vi "Explain Error (Improved) UI.vi"(8 "User VI Ref":refnum<vi>, 9 "Error Cluster":errorcluster) -> ()   [LabVIEW 2020, in "Explain Error Improved Dialog.lvlib"]
uses:
  Explain Error Improved Dialog/Explain Error Improved Dialog.lvlib
  <vilib>/Utility/error.llb/DialogTypeEnum.ctl
  <vilib>/Utility/error.llb/DialogType.ctl
  fc0d4d85-7f14-4b45-b7f8-c4820347555e.vi
  <vilib>/Platform/browser.llb/Open URL in Default Browser (string).vi
  <vilib>/Utility/inputDevices.llb/mouseAcquire.vi
  <vilib>/Utility/inputDevices.llb/keyboardAcquire.vi
  <vilib>/Utility/cursorutil.llb/Set Cursor (Icon Pict).vi
  <vilib>/Utility/inputDevices.llb/closeKeyboard.vi
  <vilib>/Utility/inputDevices.llb/closeMouse.vi
panel:
  in  "search google":bool
  out "Explanation":string
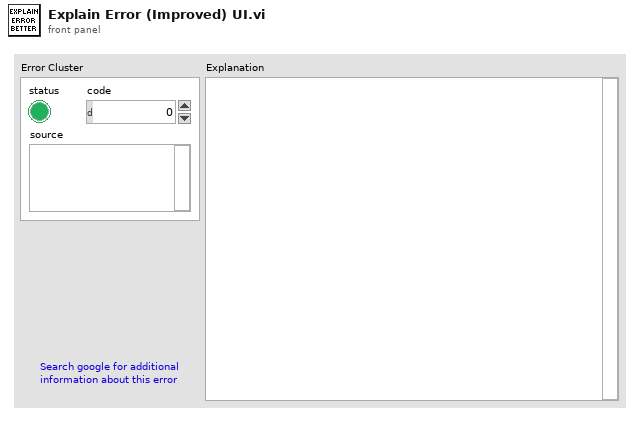
[diagram p1: front panel]
types:
  T1 = typedef "DialogTypeEnum.ctl" = enum16{"no dialog", "OK message", "continue or stop message", "auto error handling dialog", "OK message + warnings", "continue/stop + warnings"}
  T2 = typedef "DialogType.ctl" = u16
  T3 = cluster{"vi name":string, "start":i32, "end":i32}[]
  T4 = typedef "LVPoint32TypeDef.ctl" = cluster{"Horizontal":i32, "Vertical":i32}
  T5 = cluster{"button 1":bool, "button 2":bool, "button 3":bool, "button 4":bool}
  T6 = cluster{"vi name":string, "start":i32, "end":i32}
  T7 = enum16{"0", "1", "2", "3", "4", "5", "6", "7", "8", "9", "A", "B", "C", "D", "E", "F", "G", "H", "I", "J", "K", "L", "M", "N", "O", "P", "Q", "R", "S", "T", "U", "V", "W", "X", "Y", "Z", "F1", "F2", "F3", "F4", "F5", "F6", "F7", "F8", "F9", "F10", "F11", "F12", "F13", "F14", "F15", "ADD", "BACK", "BACKSLASH", "CAPITAL", "COMMA", "DECIMAL", "DELETE", "DIVIDE", "DOWN", "END", "EQUALS", "ESCAPE", "GRAVE (`)", "HOME", "INSERT", "LBRACKET", "LCONTROL", "LEFT", "L ALT", "LSHIFT", "LWIN", "MINUS", "MULTIPLY", "NEXT", "NUMLOCK", "NUMPAD_0", "NUMPAD_1", "NUMPAD_2", "NUMPAD_3", "NUMPAD_4", "NUMPAD_5", "NUMPAD_6", "NUMPAD_7", "NUMPAD_8", "NUMPAD_9", "PAUSE", "PERIOD", "PRIOR (PG UP)", "RBRACKET", "RCONTROL", "RETURN", "RIGHT", "R ALT", "RSHIFT", "RWIN", "SCROLL", "SEMICOLON", "SLASH", "SPACE", "SUBTRACT", "TAB", "UP", "ENTER (num pad)", "' (quote)"}[]
  T8 = cluster{"Shift":bool, "Ctrl":bool, "Alt":bool, "Cmd":bool, "Opt":bool}
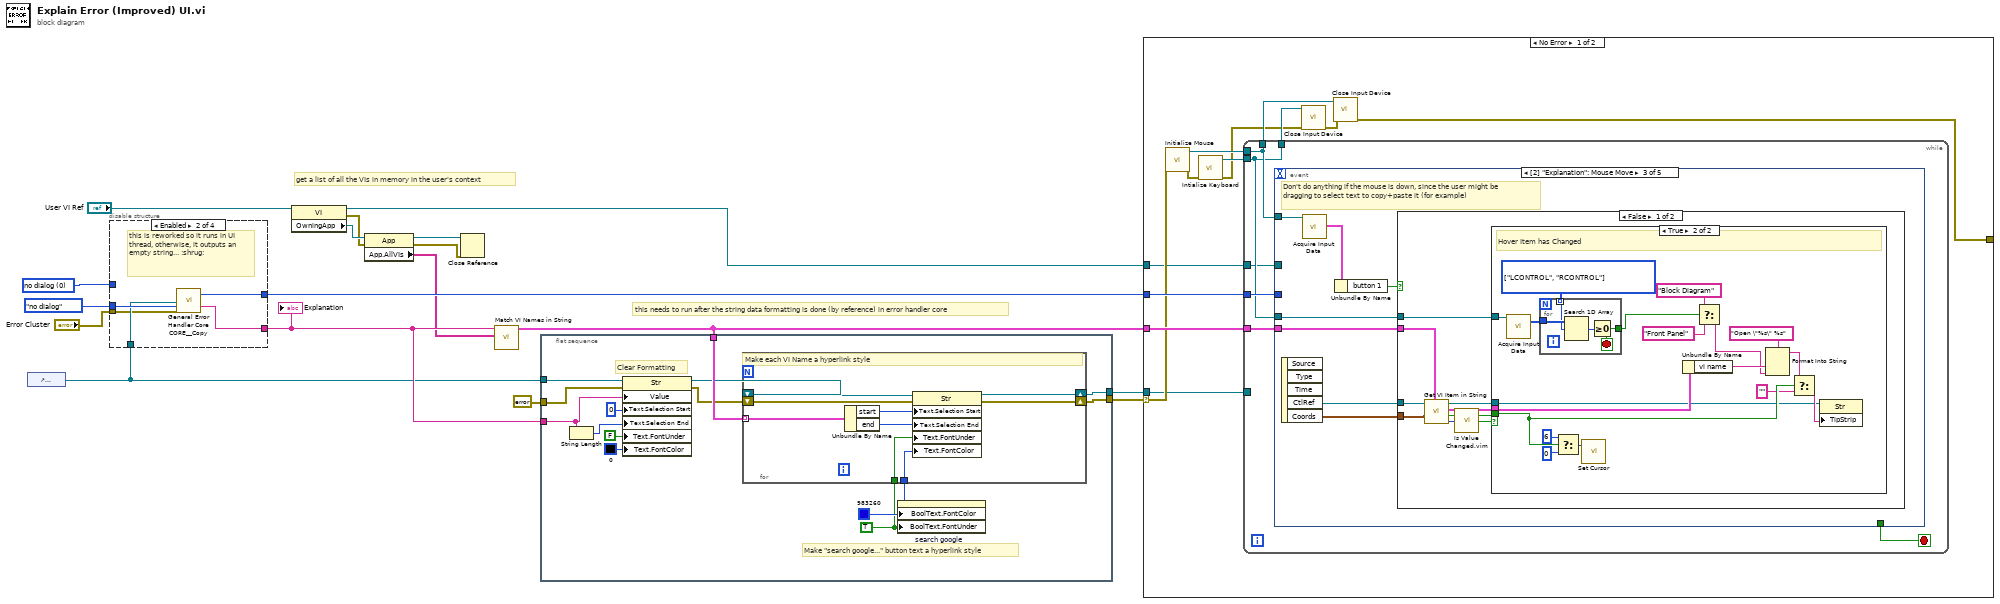
[diagram p0: block diagram]
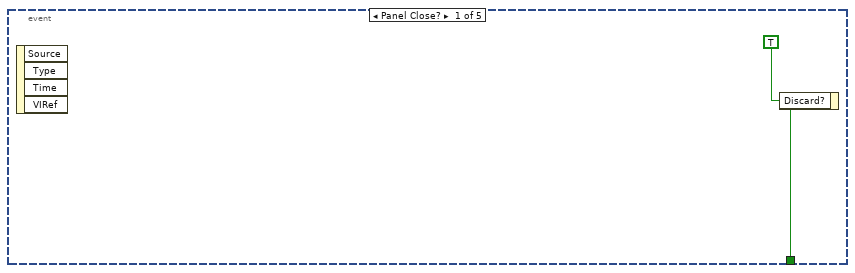
[diagram p2: hidden frame]
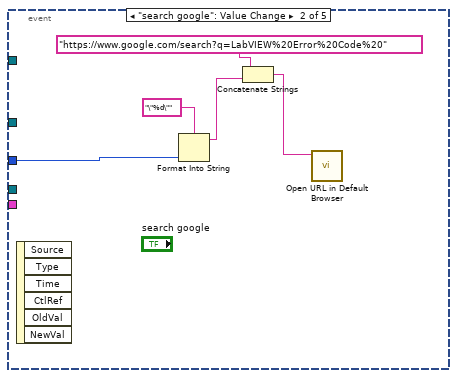
[diagram p3: hidden frame]
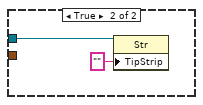
[diagram p5: hidden frame]
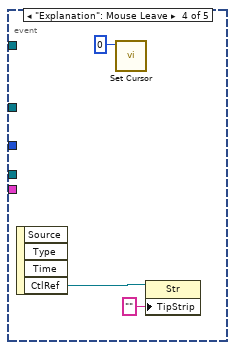
[diagram p6: hidden frame]
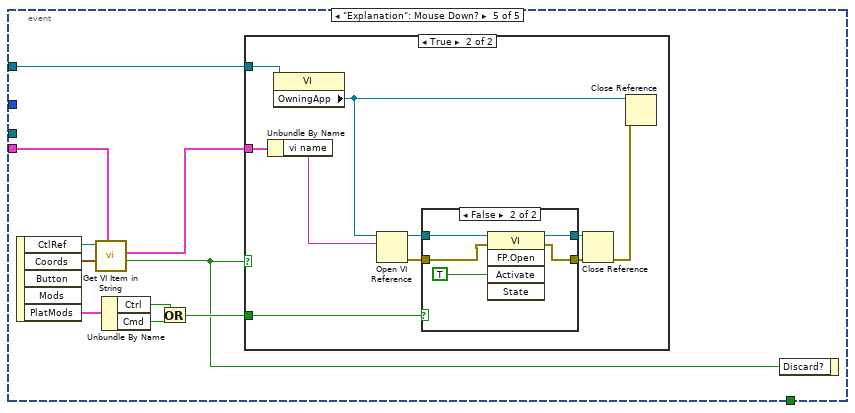
[diagram p7: hidden frame]
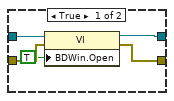
[diagram p9: hidden frame]
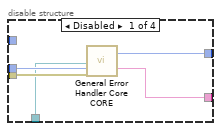
[diagram p11: hidden frame]
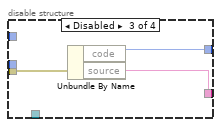
[diagram p12: hidden frame]
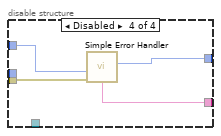
[diagram p13: hidden frame]
diagram:
  w12 = T2 0 items=["no dialog", "OK message", "continue or stop message", "OK message + warnings", "continue/stop + warnings"] ("type of dialog (OK msg:1)")
  # "this needs to run after the string data formatting is done (by reference) in error handler core"
  # "get a list of all the VIs in memory in the user's context"
  n1 = control-ref of="Explanation"() -> (w9:refnum<vi>)
  n2 = disable-structure shown="Enabled" {
    disable-tunnel: "Error Cluster" -> [w22 w23 w30 w34]
    disable-tunnel: DialogTypeEnum."no dialog" ("type of dialog (OK msg:1)") -> [w21 w27 _ _]
    disable-tunnel: [w19 w26 w28 w33] -> w10
    disable-tunnel: [w18 w25 w29 w32] -> w14
    disable-tunnel: w12 -> [_ _ _ w31]
    disable-tunnel: w9 -> [w20 w24 _ _]
    frame Disabled {
      n3 = call <vilib>:"General Error Handler Core CORE.vi"("String to Format (not a refnum)"=w20, "type of dialog (OK msg:1)"=w21, "error in (no error)"=w22) -> ("code out"=w18:i32, "message"=w19:string)  [unwired: 11 in, 4 out]
    }
    frame Enabled {
      # "this is reworked so it runs in UI thread, otherwise, it outputs an empty string... :shrug:"
      n4 = call "General Error Handler Core CORE__Copy.vi"("String to Format (not a refnum)"=w24, "type of dialog (OK msg:1)"=w27, "error in (no error)"=w23) -> ("code out"=w25:i32, "message"=w26:string)  [unwired: 11 in, 4 out]
    }
    frame Disabled {
      n5 = Unbundle By Name(w30) -> ("code"=w29:i32, "source"=w28:string)
    }
    frame Disabled {
      n6 = call <vilib>:"Simple Error Handler.vi"("type of dialog (OK msg:1)"=w31, "error in (no error)"=w34) -> ("code out"=w32:i32, "message"=w33:string)  [unwired: 3 in, 3 out]
    }
  }
  "Explanation" <- w10
  n7 = property class="VI"(reference="User VI Ref") -> (reference out=w7:refnum<vi>, error out=w3:errorcluster, "OwningApp"=w6:refnum<vi>)  [unwired: 1 in]
  n8 = property class="App"(reference=w6, error in=w3) -> (reference out=w4:refnum<vi>, error out=w2:errorcluster, "App.AllVIs"=w5:string[])
  n9 = Close Reference(reference=w4, error in (no error)=w2) -> ()  [unwired: 1 out]
  n10 = call "Match VI Names in String.vi"("Application:All VIs In Memory"=w5, "string"=w10) -> ("vi names"=w17:T3)  [unwired: 9 in]
  n11 = flat-sequence {
    tunnel: w17 -> [w48]
    tunnel: [w47] -> w16
    tunnel: w10 -> [w46]
    tunnel: w9 -> [w45]
    tunnel: [w44] -> w8
    tunnel: errorcluster {"status"=FALSE, "code"=0, "source"=""} ("error out") -> [w43]
    frame #0 {
      w38 = TRUE ("Text.Font:Underline")
      w39 = u32 983260
      # "Make \"search google...\" button text a hyperlink style"
      # "Clear Formatting"
      n12 = String Length(string=w46) -> (length=w37:i32)
      n13 = property class="Str"(reference=w45, error in=w43, "Value"=w46, "Text.Selection Start"=u32 0 ("Text.Selection:Start"), "Text.Selection End"=w37, "Text.FontUnder"=FALSE ("Text.Font:Underline"), "Text.FontColor"=u32 0 ("Text.Font:Color")) -> (reference out=w42:refnum<vi>, error out=w35:errorcluster)
      n14 = for {
        tunnel: w48 -> [w56] mode=indexing
        shift-right: [w53] -> w47
        shift-left: w42 -> [w57]
        tunnel: w39 -> [w52]
        tunnel: w38 -> [w51]
        shift-right: [w49] -> w44
        shift-left: w35 -> [w50]
        # "Make each VI Name a hyperlink style"
        n15 = Unbundle By Name(w56) -> ("start"=w55:i32, "end"=w54:i32)
        n16 = property class="Str"(reference=w57, error in=w50, "Text.Selection Start"=w55, "Text.Selection End"=w54, "Text.FontUnder"=w51, "Text.FontColor"=w52) -> (reference out=w53:refnum<vi>, error out=w49:errorcluster)
      }
      n17 = property on="search google" class="Bool (strict)"("BoolText.FontColor"=w39, "BoolText.FontUnder"=w38) -> ()  [unwired: 2 in, 2 out]
    }
  }
  n18 = case shown="No Error" w8 {
    selector: w8 -> [w64 w156]
    tunnel: w17 -> [w70 _]
    tunnel: w16 -> [w58 _]
    tunnel: w14 -> [w65 _]
    tunnel: [w59 w156] -> _
    tunnel: w7 -> [w60 _]
    frame No Error {
      n19 = call <vilib>:"Initialize Mouse.vi"("error in (no error)"=w64) -> ("error out"=w63:errorcluster, "device ID"=w69:refnum<k1>)  [unwired: 9 in]
      n20 = call <vilib>:"Intialize Keyboard.vi"("error in (no error)"=w63) -> ("error out"=w62:errorcluster, "device ID"=w67:refnum<k1>)  [unwired: 9 in]
      n21 = while {
        tunnel: w70 -> [w75]
        tunnel: w69 -> [w74]
        tunnel: [w74] -> w68
        tunnel: w58 -> [_]
        tunnel: w65 -> [w73]
        tunnel: w67 -> [w72]
        tunnel: [w72] -> w66
        tunnel: w60 -> [w71]
        stop <- w76 stop-if-true
        n22 = event shown="[2] \"Explanation\": Mouse Move" {
          selector: _ -> [_ _ _ _ _]
          dyn-events: _ -> [_ _ _ _ _]
          timeout: _ -> [_ _ _ _ _]
          tunnel: [w77 _ _ _ _] -> w76
          tunnel: w75 -> [_ _ w88 _ w134]
          tunnel: w74 -> [_ _ w86 _ _]
          tunnel: w73 -> [_ w82 _ _ _]
          tunnel: w72 -> [_ _ w83 _ _]
          tunnel: w71 -> [_ _ _ _ w127]
          event Panel Close? {
            w77 = TRUE ("Discard?")
            n23 = event-data() -> ()  [unwired: 1 in, 4 out]
            n24 = event-data("Discard?"=w77) -> ()  [unwired: 1 in, 1 out]
          }
          event "search google": Value Change {
            n25 = event-data() -> ()  [unwired: 1 in, 6 out]
            n26 = Format Into String(format string="\"%d\"", w82) -> (resulting string=w81:string)  [unwired: 2 in, 1 out]
            n27 = Concatenate Strings("https://www.google.com/search?q=LabVIEW%20Error%20Code%20" ("format string"), w81) -> (w79:string)
            n28 = call-poly <vilib>:"Open URL in Default Browser.vi"("URL"=w79) -> ()  [unwired: 5 in, 2 out]
          }
          event "Explanation": Mouse Move {
            # "Don't do anything if the mouse is down, since the user might be dragging to select text to copy+paste it (for example)"
            n29 = event-data() -> ("CtlRef"=w87:refnum<vi>, "Coords"=w89:T4)  [unwired: 1 in, 3 out]
            n30 = call-poly <vilib>:"Acquire Input Data.vi"("device ID"=w86) -> ("button info"=w85:T5)  [unwired: 15 in, 3 out]
            n31 = Unbundle By Name(w85) -> ("button 1"=w84:bool)
            n32 = case shown="False" w84 {
              tunnel: w89 -> [w98 _]
              tunnel: w88 -> [w97 _]
              tunnel: w87 -> [w94 w122]
              tunnel: w83 -> [w93 _]
              frame False {
                n33 = call "Get VI Item in String.vi"("items"=w97, "Coords"=w98, "String in"=w94) -> ("item index"=w91:i32, "active item"=w95:bool, "item at coords"=w96:T6, "String out"=w92:refnum<vi>)  [unwired: 5 in]
                n34 = call "Is Value Changed.vim"("value"=w91) -> ("changed or first call?"=w90:bool)
                n35 = case shown="True" w90 {
                  tunnel: w96 -> [_ w112]
                  tunnel: w95 -> [_ w101]
                  tunnel: w93 -> [_ w109]
                  tunnel: w92 -> [_ w99]
                  frame False {
                  }
                  frame True {
                    w108 = T7 [enum."LCONTROL", enum."RCONTROL"] items=["0", "1", "2", "3", "4", "5", "6", "7", "8", "9", "A", "B", "C", "D", "E", "F", "G", "H", "I", "J", "K", "L", "M", "N", "O", "P", "Q", "R", "S", "T", "U", "V", "W", "X", "Y", "Z", "F1", "F2", "F3", "F4", "F5", "F6", "F7", "F8", "F9", "F10", "F11", "F12", "F13", "F14", "F15", "ADD", "BACK", "BACKSLASH", "CAPITAL", "COMMA", "DECIMAL", "DELETE", "DIVIDE", "DOWN", "END", "EQUALS", "ESCAPE", "GRAVE (`)", "HOME", "INSERT", "LBRACKET", "LCONTROL", "LEFT", "L ALT", "LSHIFT", "LWIN", "MINUS", "MULTIPLY", "NEXT", "NUMLOCK", "NUMPAD_0", "NUMPAD_1", "NUMPAD_2", "NUMPAD_3", "NUMPAD_4", "NUMPAD_5", "NUMPAD_6", "NUMPAD_7", "NUMPAD_8", "NUMPAD_9", "PAUSE", "PERIOD", "PRIOR (PG UP)", "RBRACKET", "RCONTROL", "RETURN", "RIGHT", "R ALT", "RSHIFT", "RWIN", "SCROLL", "SEMICOLON", "SLASH", "SPACE", "SUBTRACT", "TAB", "UP", "ENTER (num pad)", "' (quote)"] ("keys pressed")
                    # "Hover Item has Changed"
                    n36 = call-poly <vilib>:"Acquire Input Data.vi"("device ID"=w109) -> ("keys pressed"=w107:T7)  [unwired: 16 in, 2 out]
                    n37 = for {
                      tunnel: w108 -> [w119] mode=indexing
                      tunnel: w107 -> [w120]
                      tunnel: [w117] -> w106
                      stop <- w117 stop-if-true
                      n38 = Search 1D Array(1D array=w120, element=w119) -> (index of element=w118:i32)  [unwired: 1 in]
                      n39 = Greater Or Equal To 0?(x=w118) -> (x >= 0?=w117:bool)
                    }
                    n40 = Select(t=u16 6 ("icon"), s=w101, f=u16 0 ("icon")) -> (s? t:f=w114:u16)
                    n41 = call-poly <vilib>:"Set Cursor.vi"("icon"=w114) -> ()  [unwired: 9 in, 2 out]
                    n42 = Unbundle By Name(w112) -> ("vi name"=w111:string)
                    n43 = Select(t="Block Diagram" ("format string"), s=w106, f="Front Panel" ("format string")) -> (s? t:f=w103:string)
                    n44 = Format Into String(format string="Open \"%s\" %s", w111, w103) -> (resulting string=w102:string)  [unwired: 2 in, 1 out]
                    n45 = Select(t=w102, s=w101, f="" ("format string")) -> (s? t:f=w113:string)
                    n46 = property class="Str"(reference=w99, "TipStrip"=w113) -> ()  [unwired: 1 in, 2 out]
                  }
                }
              }
              frame True {
                n47 = property class="Str"(reference=w122, "TipStrip"="" ("Tip Strip")) -> ()  [unwired: 1 in, 2 out]
              }
            }
          }
          event "Explanation": Mouse Leave {
            n48 = event-data() -> ("CtlRef"=w123:refnum<vi>)  [unwired: 1 in, 3 out]
            n49 = call-poly <vilib>:"Set Cursor.vi"("icon"=u16 0) -> ()  [unwired: 9 in, 2 out]
            n50 = property class="Str"(reference=w123, "TipStrip"="" ("Tip Strip")) -> ()  [unwired: 1 in, 2 out]
          }
          event "Explanation": Mouse Down? {
            n51 = event-data() -> ("CtlRef"=w133:refnum<vi>, "Coords"=w135:T4, "PlatMods"=w132:T8)  [unwired: 1 in, 2 out]
            n52 = call "Get VI Item in String.vi"("items"=w134, "Coords"=w135, "String in"=w133) -> ("active item"=w128:bool, "item at coords"=w126:T6)  [unwired: 5 in, 2 out]
            n53 = Unbundle By Name(w132) -> ("Ctrl"=w130:bool, "Cmd"=w131:bool)
            n54 = Or(x=w130, y=w131) -> (x .or. y?=w129:bool)
            n55 = case shown="True" w128 {
              tunnel: w129 -> [_ w141]
              tunnel: w127 -> [_ w138]
              tunnel: w126 -> [_ w140]
              frame False {
              }
              frame True {
                n56 = Unbundle By Name(w140) -> ("vi name"=w139:string)
                n57 = property class="VI"(reference=w138) -> ("OwningApp"=w137:refnum<vi>)  [unwired: 1 in, 2 out]
                n58 = Open VI Reference(application reference (local)=w137, vi path=w139) -> (vi reference=w145:refnum<vi>, error out=w144:errorcluster)  [unwired: 4 in]
                n59 = case shown="False" w141 {
                  tunnel: w145 -> [w150 w155]
                  tunnel: w144 -> [w149 w153]
                  tunnel: [w147 w152] -> w143
                  tunnel: [w146 w151] -> w142
                  frame True {
                    n60 = property class="VI"(reference=w150, error in=w149, "BDWin.Open"=TRUE ("Block Diagram Window:Open")) -> (reference out=w146:refnum<vi>, error out=w147:errorcluster)
                  }
                  frame False {
                    n61 = invoke class="VI" method="FP.Open"(reference=w155, error in=w153, "Activate"=TRUE ("Activate?")) -> (reference out=w151:refnum<vi>, error out=w152:errorcluster)  [unwired: 2 in, 3 out]
                  }
                }
                n62 = Close Reference(reference=w142, error in (no error)=w143) -> (error out=w136:errorcluster)
                n63 = Close Reference(reference=w137, error in (no error)=w136) -> ()  [unwired: 1 out]
              }
            }
            n64 = event-data("Discard?"=w128) -> ()  [unwired: 1 in, 1 out]
          }
        }
      }
      n65 = call-poly <vilib>:"Close Input Device.vi"("error in (no error)"=w62, "device ID"=w66) -> ("error out"=w61:errorcluster)  [unwired: 8 in]
      n66 = call-poly <vilib>:"Close Input Device.vi"("error in (no error)"=w61, "device ID"=w68) -> ("error out"=w59:errorcluster)  [unwired: 8 in]
    }
    frame Error {
    }
  }
